vi "Running State.vi"(1 "Reset? (F)":bool) -> (0 "Running?":bool)   [LabVIEW 2018, in "GLog.lvlib" / "UI Updater.lvlib"]
uses:
  UI Updater.lvlib
panel:
  # "Connector Pane"
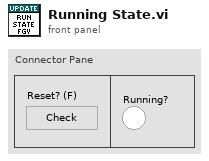
[diagram p1: front panel]
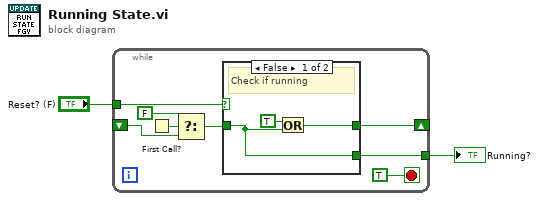
[diagram p0: block diagram]
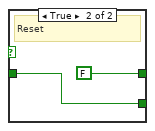
[diagram p2: hidden frame]
diagram:
  n1 = while {
    shift-right: [w9] -> _
    shift-left: _ -> [w4]
    tunnel: "Reset? (F)" -> [w8]
    tunnel: [w7] -> w2
    stop <- TRUE stop-if-true
    n2 = First Call?() -> (First Call?: T/F=w6:bool)
    n3 = Select(t=FALSE, s=w6, f=w4) -> (s? t:f=w3:bool)
    n4 = case shown="False" w8 {
      tunnel: [w11 FALSE] -> w9
      tunnel: w3 -> [w13 w15]
      tunnel: [w13 w15] -> w7
      frame False {
        # "Check if running"
        n5 = Or(x=TRUE, y=w13) -> (x .or. y?=w11:bool)
      }
      frame True {
        # "Reset"
      }
    }
  }
  "Running?" <- w2
